vi "BB from Refnum.vi"(3 "BB Refnum":T1 {"refnum" format="%.0x"}) -> (5 "BB U64":u64)   [LabVIEW 2021, in "Iceoryx.lvlib"]
uses:
  Iceoryx.lvlib
  Typedef/BB Refnum.ctl
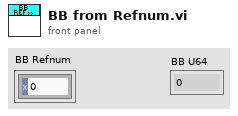
[diagram p1: front panel]
types:
  T1 = typedef "Iceoryx.lvlib/BB Refnum.ctl" = cluster{"refnum":u64, "BB":enum8{"bb"}}
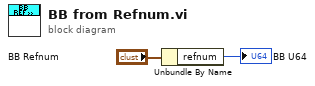
[diagram p0: block diagram]
diagram:
  n1 = Unbundle By Name("BB Refnum") -> ("refnum"=→"BB U64":u64)
